vi "Divide in Squares.vi"(6 "Offset (0)":i16, 8 "Border (2)":i16=2, 9 "Width (48)":i16=48, 10 "Coords":T1={"Horizontal"=-10000, "Vertical"=-10000}, 11 "Rectangle":T2) -> (0 "Column":i32, 1 "Row":i32, 2 "in squares?":bool, 3 "Zones Rectangles":T3(array[cluster]))   [LabVIEW 2012]
doc: "Creates an array of squares based on the width and border parameters.\n\nIf coordinates are supplied, the VI also calculates in which row & column the coordinates are pointing. \n\n-1: outside of all squares (can be in-between squares or outside)\n\nThis VI could be used to create a grid to snap objects in pre-defined patterns."
uses:
  <vilib>/Utility/miscctls.llb/LVPoint32TypeDef.ctl
panel:
  # "Rectangle"
  # "Offset"
  # "border"
  # "border"
  # "Offset"
  # "Width"
  # "Width"
  # "border"
  # "border"
  # "Width"
  # "Width"
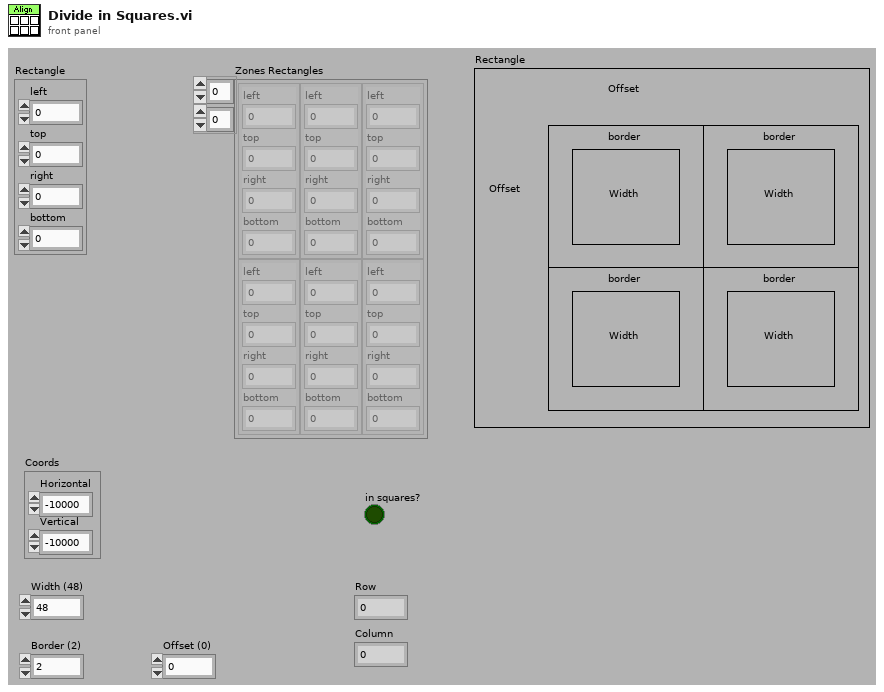
[diagram p1: front panel]
types:
  T1 = typedef "LVPoint32TypeDef.ctl" = cluster{"Horizontal":i32, "Vertical":i32}
  T2 = cluster{"left":i16, "top":i16, "right":i16, "bottom":i16}
  T3 = cluster{"left":i16, "top":i16, "right":i16, "bottom":i16}[][]
  T4 = cluster{"left":i16, "top":i16, "right":i16, "bottom":i16}[]
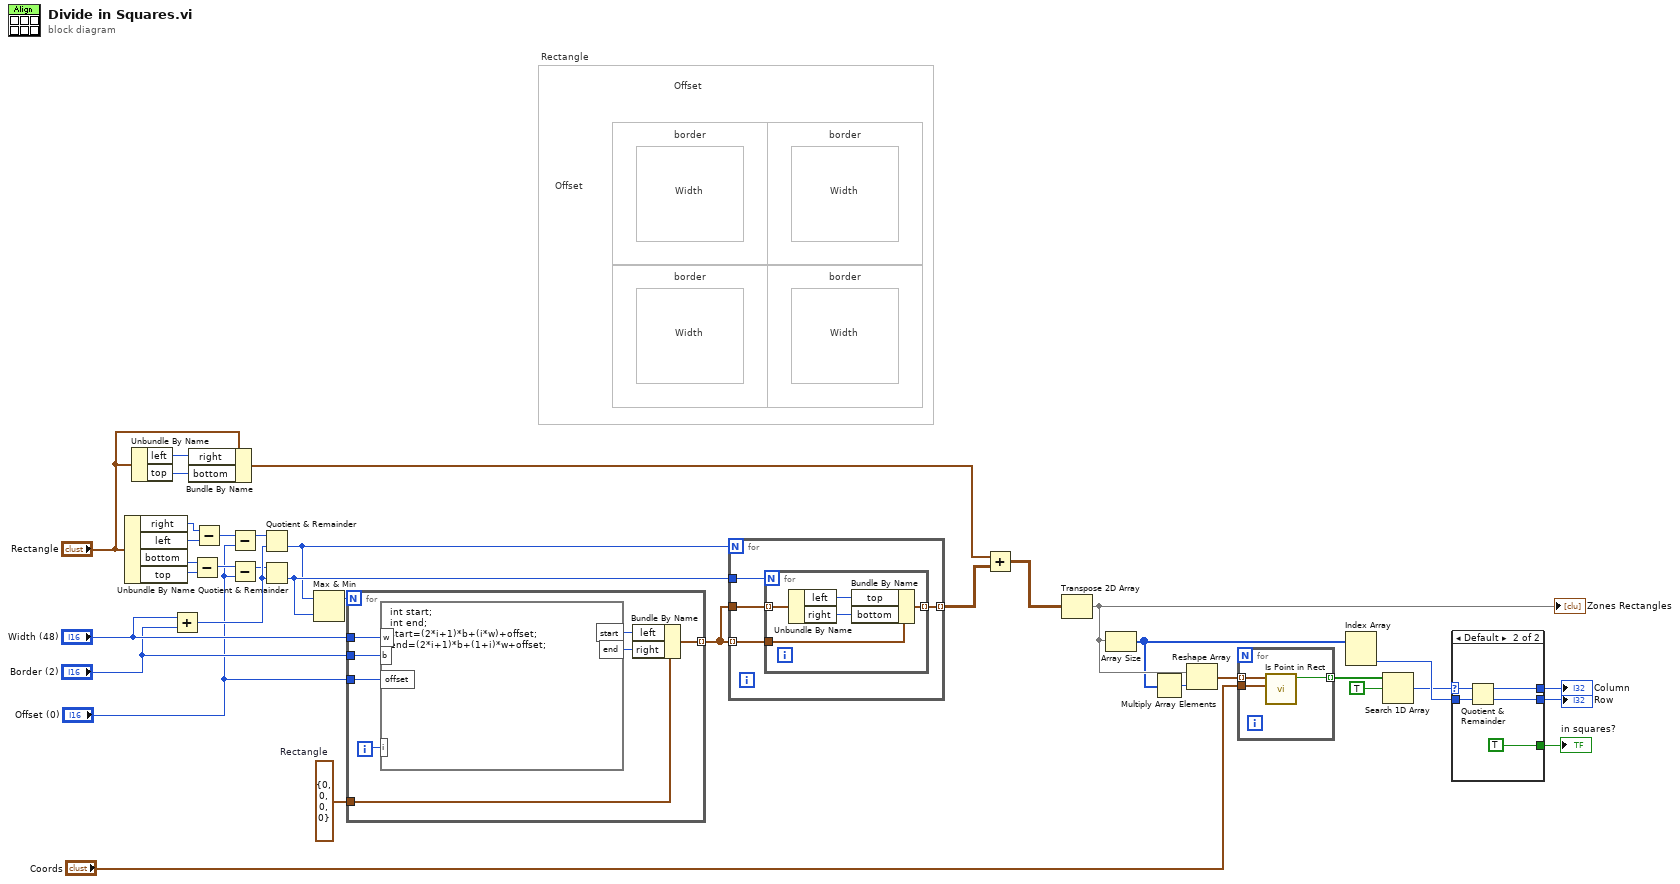
[diagram p0: block diagram]
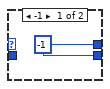
[diagram p2: hidden frame]
diagram:
  w26 = T2 {"left"=0, "top"=0, "right"=0, "bottom"=0}  # Rectangle
  # "Width"
  # "border"
  # "Width"
  # "border"
  # "Width"
  # "border"
  # "Offset"
  # "Offset"
  # "Width"
  # "border"
  # "Rectangle"
  n1 = Unbundle By Name("Rectangle") -> ("right"=w22:i16, "left"=w34:i16, "bottom"=w20:i16, "top"=w21:i16)
  n2 = Unbundle By Name("Rectangle") -> ("left"=w11:i16, "top"=w10:i16)
  n3 = Add(x="Width (48)", y="Border (2)") -> (x+y=w30:i16)
  n4 = Bundle By Name(cluster="Rectangle", "right"=w11, "bottom"=w10) -> (w6:T2)
  n5 = Subtract(x=w20, y=w21) -> (x-y=w3:i16)
  n6 = Subtract(x=w22, y=w34) -> (x-y=w5:i16)
  n7 = Subtract(x=w5, y="Offset (0)") -> (x-y=w4:i16)
  n8 = Subtract(x=w3, y="Offset (0)") -> (x-y=w1:i16)
  n9 = Quotient & Remainder(x=w4, y=w30) -> (floor(x/y)=w23:i16)  [unwired: 1 out]
  n10 = Quotient & Remainder(x=w1, y=w30) -> (floor(x/y)=w24:i16)  [unwired: 1 out]
  n11 = Max & Min(x=w23, y=w24) -> (max(x,y)=w27:i16)  [unwired: 1 out]
  n12 = for {
    N: w27 -> [_]
    tunnel: "Width (48)" -> [w43]
    tunnel: "Border (2)" -> [w42]
    tunnel: w26 -> [w40]
    tunnel: [w39] -> w25 mode=indexing
    tunnel: "Offset (0)" -> [w36]
    i -> [w41]
    n13 = formula code="int start;\nint end;\nstart=(2*i+1)*b+(i*w)+offset;\nend=(2*i+1)*b+(1+i)*w+offset;"("w"=w43, "b"=w42, "i"=w41, "offset"=w36) -> ("start"=w38:i32, "end"=w37:i32)
    n14 = Bundle By Name(cluster=w40, "left"=w38, "right"=w37) -> (w39:T2)
  }
  n15 = for {
    N: w23 -> [_]
    tunnel: w24 -> [w47]
    tunnel: [w46] -> w8 mode=indexing
    tunnel: w25 -> [w45] mode=indexing
    tunnel: w25 -> [w44]
    n16 = for {
      N: w47 -> [_]
      tunnel: [w52] -> w46 mode=indexing
      tunnel: w45 -> [w51]
      tunnel: w44 -> [w50] mode=indexing
      n17 = Unbundle By Name(w50) -> ("left"=w49:i16, "right"=w48:i16)
      n18 = Bundle By Name(cluster=w51, "top"=w49, "bottom"=w48) -> (w52:T2)
    }
  }
  n19 = Add(x=w6, y=w8) -> (x+y=w7:T3)
  n20 = Transpose 2D Array(2D array=w7) -> (transposed array=w16:T3)
  "Zones Rectangles" <- w16
  n21 = Array Size(array=w16) -> (size(s)=w13:i32[])
  n22 = Multiply Array Elements(1:w13) -> (0:w19:i32)
  n23 = Reshape Array(w16, w19) -> (w33:T4)
  n24 = for {
    tunnel: w33 -> [w55] mode=indexing
    tunnel: "Coords" -> [w54]
    tunnel: [w53] -> w31 mode=indexing
    n25 = call "Is Point in Rect.vi"("point"=w54, "rect"=w55) -> ("Point in Rect?"=w53:bool)  [unwired: 9 out]
  }
  n26 = Index Array(array=w13) -> (element #2=w15:i32)  [unwired: 2 in, 1 out]
  n27 = Search 1D Array(1D array=w31, element=TRUE) -> (index of element=w14:i32)  [unwired: 1 out]
  n28 = case shown="Default" w14 {
    selector: w14 -> [_ w58]
    tunnel: [w56 w61] -> w18
    tunnel: [w56 w60] -> w17
    tunnel: w15 -> [_ w59]
    tunnel: [_ TRUE] -> w12
    frame -1 {
      w56 = -1
    }
    frame Default {
      n29 = Quotient & Remainder(x=w58, y=w59) -> (x-y*floor(x/y)=w61:i32, floor(x/y)=w60:i32)
    }
  }
  "Column" <- w18
  "Row" <- w17
  "in squares?" <- w12
